vi "Check if Feed is Registered.vi"(8 "error in":errorcluster, 11 "feed URI":string) -> (0 "error out":errorcluster, 1 "feed name":string, 2 "feed URI registered?":bool, 3 "feed URI out":string)   [LabVIEW 2014, in "NIPM_API.lvlib"]
doc: "Checks if the feed URI is currently registered in NI Package Manager on this computer\n\nINPUT(s)\n<b>Feed URI:</b> Specifies the location of the feed (e.g. network folder, web server, etc)\n\nOUTPUT(s)\n<b>Feed URI out:</b> Outputs the specified feed URI\n\n<b>Feed URI registered?:</b> Outputs whether the specified feed URI is registered on this computer\n\n<b>Feed name:</b> Outputs the name of the feed, if the specified feed URI is registered on this computer"
uses:
  NIPM_API.lvlib
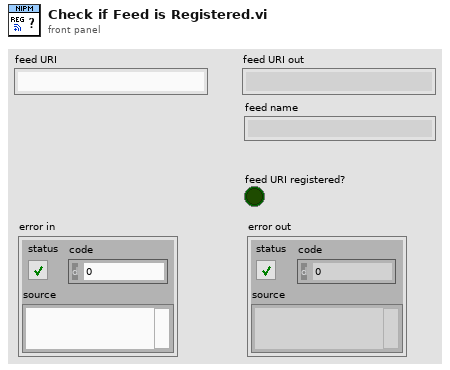
[diagram p1: front panel]
types:
  T1 = typedef "NIPM_API.lvlib/feed.ctl" = cluster{"Name":string, "URI":string}
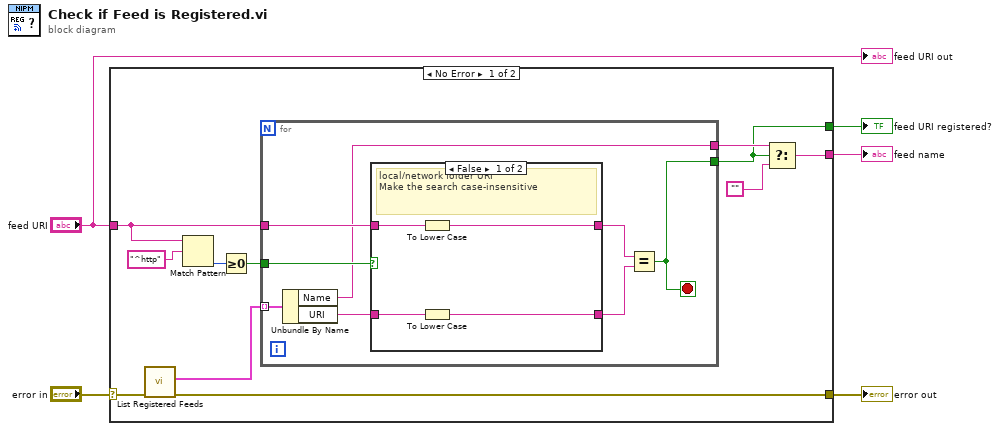
[diagram p0: block diagram]
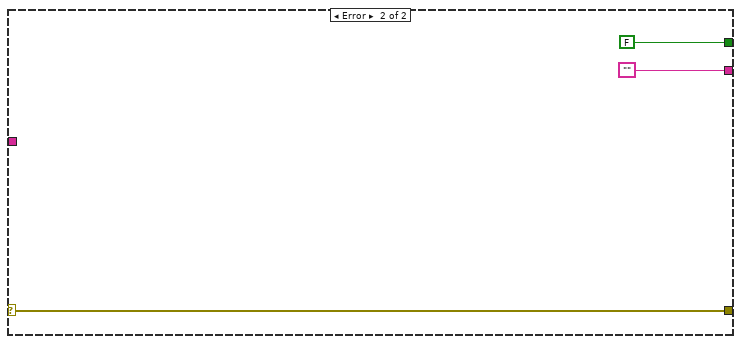
[diagram p3: hidden frame]
diagram:
  n1 = case shown="No Error" "error in" {
    selector: "error in" -> [w16 w33]
    tunnel: [w15 w33] -> w4
    tunnel: "feed URI" -> [w11 _]
    tunnel: [w6 FALSE] -> w2
    tunnel: [w7 ""] -> w1
    frame No Error {
      n2 = call "List Registered Feeds.vi"("error in"=w16) -> ("error out"=w15:errorcluster, "registered feeds"=w14:T1[])  [unwired: 9 in]
      n3 = Match Pattern(string=w11, regular expression="^http") -> (offset past match=w12:i32)  [unwired: 1 in, 3 out]
      n4 = Greater Or Equal To 0?(x=w12) -> (x >= 0?=w10:bool)
      n5 = for {
        tunnel: w14 -> [w24] mode=indexing
        tunnel: w11 -> [w20]
        tunnel: w10 -> [w23]
        tunnel: [w17] -> w9
        tunnel: [w18] -> w6
        stop <- w18 stop-if-true
        n6 = Unbundle By Name(w24) -> ("Name"=w17:string, "URI"=w22:string)
        n7 = case shown="False" w23 {
          tunnel: [w27 w30] -> w19
          tunnel: w20 -> [w28 w30]
          tunnel: [w25 w29] -> w21
          tunnel: w22 -> [w26 w29]
          frame False {
            # "local/network folder URI\nMake the search case-insensitive"
            n8 = To Lower Case(string=w28) -> (all lower case string=w27:string)
            n9 = To Lower Case(string=w26) -> (all lower case string=w25:string)
          }
          frame True {
            # "http URI \nMake the search case-sensitive"
          }
        }
        n10 = Equal?(x=w19, y=w21) -> (x = y?=w18:bool)
      }
      n11 = Select(t=w9, s=w6, f="") -> (s? t:f=w7:string)
    }
    frame Error {
    }
  }
  "error out" <- w4
  "feed URI registered?" <- w2
  "feed name" <- w1
  "feed URI out" <- "feed URI"
